vi "Write.vi"(8 "error in (no error)":errorcluster, 10 "data in":dbl, 11 "DAQNavi_AO in":refnum<class "DAQNavi_AO.lvclass">) -> (0 "error out":errorcluster, 3 "DAQNavi_AO out":refnum<class "DAQNavi_AO.lvclass">)   [LabVIEW 2021, in "DAQNavi_AO.lvclass"]
uses:
  DAQNavi_AO.lvclass
  DAQNavi_AO.lvclass/DAQNavi_AO.ctl
  <userlib>/DAQNavi Polymorphic VI/write/DAQNavi Write (Analog DBL 1Chan 1Samp).vi
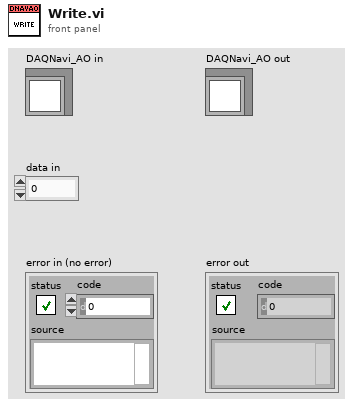
[diagram p1: front panel]
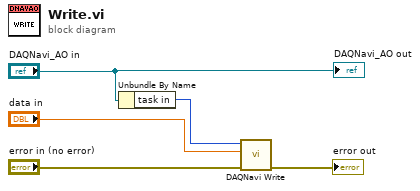
[diagram p0: block diagram]
diagram:
  n1 = Unbundle By Name("DAQNavi_AO in") -> ("task in"=w5:i32)
  n2 = call-poly <userlib>:"DAQNavi Write.vi"("error in (no error)"="error in (no error)", "data"="data in", "task in"=w5) -> ("error out"=→"error out":errorcluster)  [unwired: 6 in, 2 out]
  "DAQNavi_AO out" <- "DAQNavi_AO in"
